vi "VIH UI - Controller for Property Pages.vi"(6 "cmd (update)":T2(ring)=enum."Update", 7 "SubPanel":refnum<vi>, 8 "error in":errorcluster, 9 "Params":string[](array[string]), 10 "Item Type":T3, 11 "Project Tree":T1) -> (0 "error out":errorcluster, 3 "dup Tree Refnum":T1)   [LabVIEW 2014]
doc: "::: VI Helpeks :::\nCopyright (c) 2000-2026 Konstantin Shifershteyn. All rights reserved."
uses:
  _VIH Project Manager.llb/VIH Project Tree Typedef - Tree Item Type.ctl
  _VIH Project Manager.llb/VIH Project Tree Typedef - Tree Refnum.ctl
  VIH UI Typedef - Property Page ExtCommand.ctl
panel:
  # "VI Helpeks\nCopyright (c) 2012-2026 Konstantin Shifershteyn"
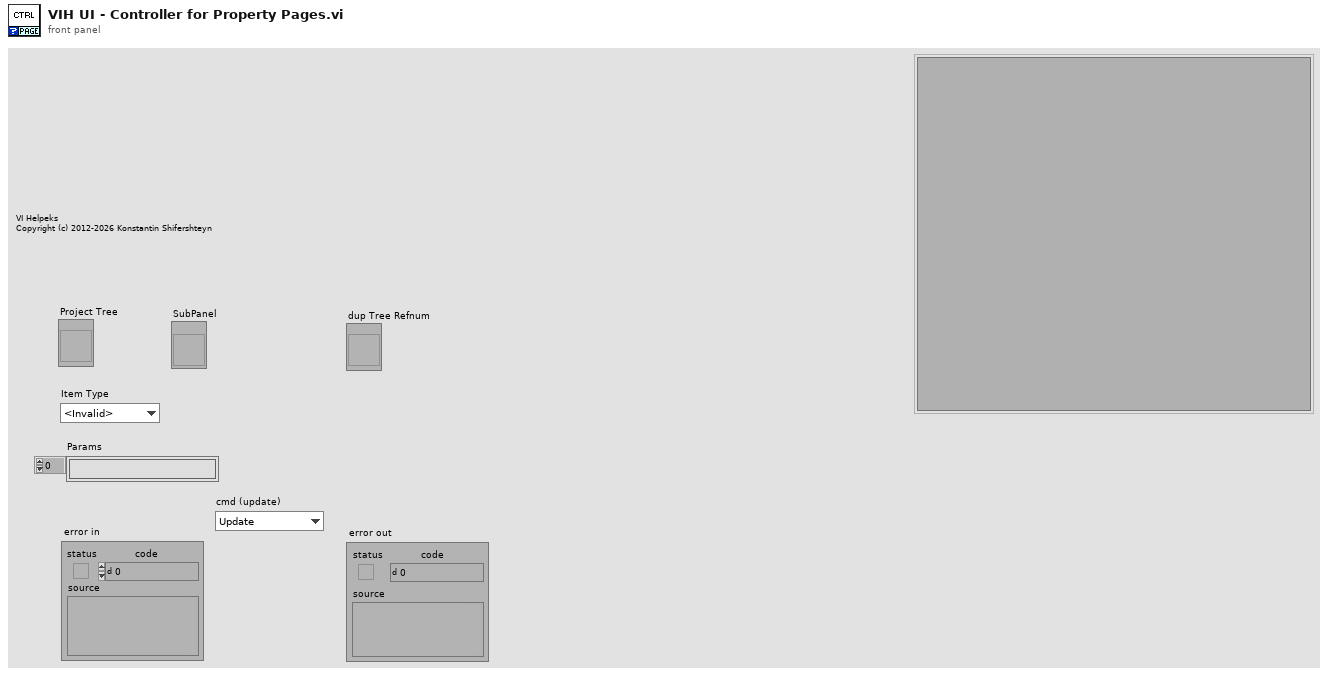
[diagram p1: front panel]
types:
  T1 = typedef "VIH Project Tree Typedef - Tree Refnum.ctl" = refnum<vi>
  T2 = enum16{"Open", "Close", "Update", "Set Category"}
  T3 = typedef "VIH Project Tree Typedef - Tree Item Type.ctl" = enum32{"<Invalid>", "Project", "Proj Files", "Proj Rules", "File Group", "Rule Group", "Any File", "LV Func", ".mnu", ".mnu (dyn)", ".vi", ".vi (dyn)", ".vit", ".vit (dyn)", ".ctl", ".ctl (dyn)", ".ctt", ".ctt (dyn)", "polyVI", "polyVI (dyn)", "expVI", "expVI (dyn)", "HTML", "PolyVI Inst"}
  T4 = typedef "VIH UI Typedef - Property Page ExtCommand.ctl" = cluster{"Action":string, "Project Tree":T1, "Params":string[]}
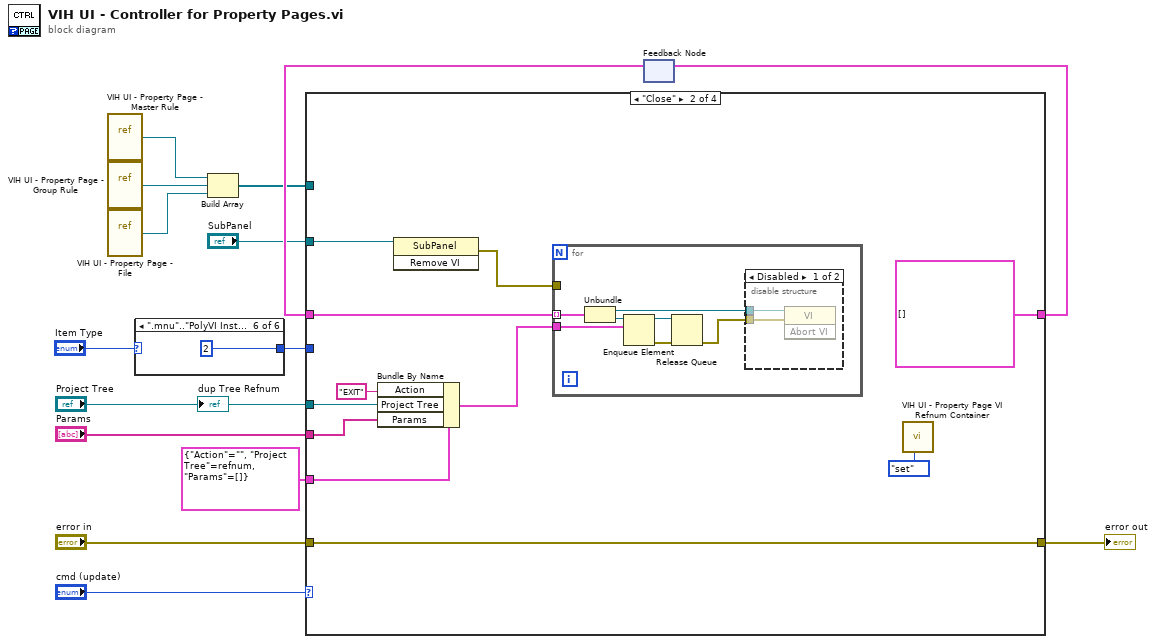
[diagram p0: block diagram]
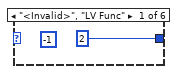
[diagram p2: hidden frame]
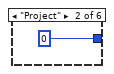
[diagram p3: hidden frame]
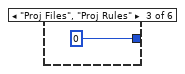
[diagram p4: hidden frame]
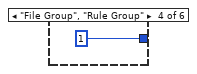
[diagram p5: hidden frame]
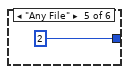
[diagram p6: hidden frame]
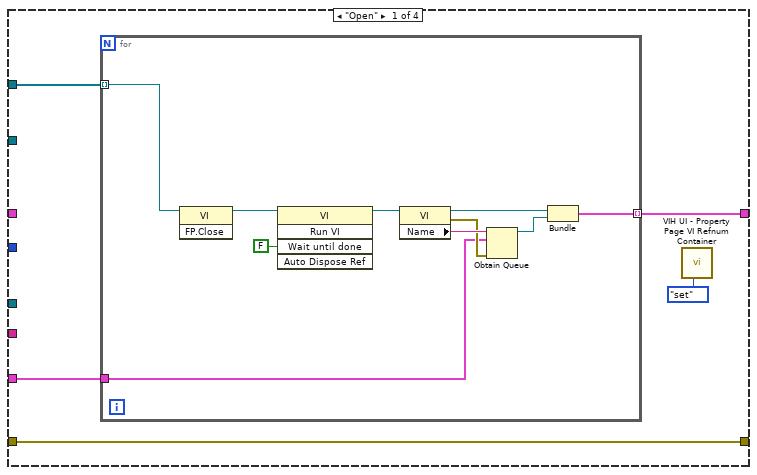
[diagram p7: hidden frame]
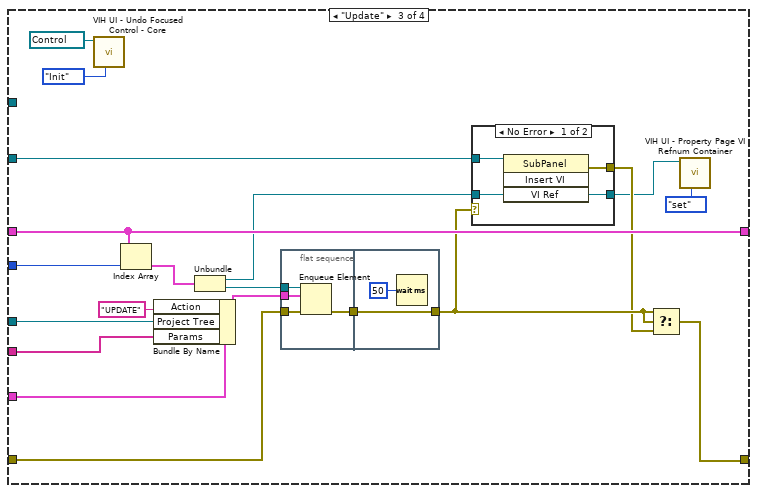
[diagram p9: hidden frame]
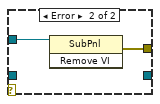
[diagram p10: hidden frame]
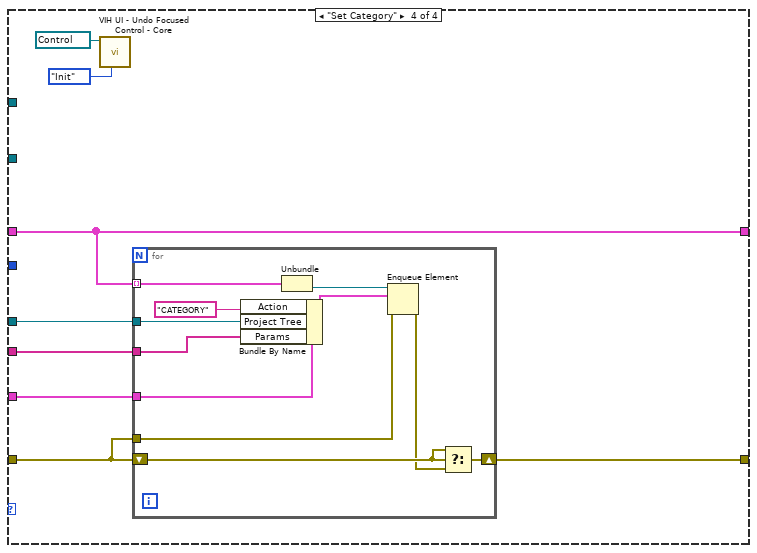
[diagram p11: hidden frame]
diagram:
  n1 = vi-ref "VIH UI - Property Page - Master Rule.vi"() -> (w7:refnum<vi>)
  n2 = vi-ref "VIH UI - Property Page - Group Rule.vi"() -> (w6:refnum<vi>)
  n3 = vi-ref "VIH UI - Property Page - File.vi"() -> (w5:refnum<vi>)
  n4 = case shown="\".mnu\"..\"PolyVI Inst\"" "Item Type" {
    tunnel: [2 0 0 1 2 2] -> w4
    frame "<Invalid>", "LV Func" {
      (unwired) -1
    }
    frame "Project" {
    }
    frame "Proj Files", "Proj Rules" {
    }
    frame "File Group", "Rule Group" {
    }
    frame "Any File" {
    }
    frame ".mnu".."PolyVI Inst" {
    }
  }
  n5 = Build Array(w7, w6, w5) -> (w2:refnum<vi>[])
  n6 = feedback #1() -> (w13:cluster{refnum<vi>, "queue out":refnum<queue>}[])  [unwired: 1 in]
  n7 = case shown="\"Close\"" "cmd (update)" {
    tunnel: [w26 cluster{refnum<vi>, "queue out":refnum<queue>}[] [] w76 w92] -> w14
    tunnel: w13 -> [_ w47 w76 w92]
    tunnel: "Params" -> [_ w42 w73 w95]
    tunnel: w4 -> [_ _ w70 _]
    tunnel: "error in" -> [w25 w46 w68 w91]
    tunnel: [w25 w46 w61 w90] -> w10
    tunnel: T4 {"Action"="", "Project Tree"=refnum, "Params"=[]} -> [w24 w45 w67 w94]
    tunnel: "Project Tree" -> [_ w43 w66 w93]
    tunnel: w2 -> [w23 _ _ _]
    tunnel: "SubPanel" -> [_ w39 w64 _]
    frame "Open" {
      n8 = for {
        tunnel: [w31] -> w26 mode=indexing
        tunnel: w24 -> [w29]
        tunnel: w23 -> [w28] mode=indexing
        n9 = invoke class="VI" method="FP.Close"(reference=w28) -> (reference out=w27:refnum<vi>)  [unwired: 2 in, 2 out]
        n10 = invoke class="VI" method="Run VI"(reference=w27, "Wait until done"=FALSE ("Wait Until Done")) -> (reference out=w35:refnum<vi>)  [unwired: 3 in, 4 out]
        n11 = property class="VI"(reference=w35) -> (reference out=w33:refnum<vi>, error out=w30:errorcluster, "Name"=w34:string)  [unwired: 1 in]
        n12 = Obtain Queue(name (unnamed)=w34, element data type=w29, error in (no error)=w30) -> (queue out=w32:refnum<queue>)  [unwired: 2 in, 2 out]
        n13 = Bundle(w33, "queue out"=w32) -> (w31:cluster{refnum<vi>, "queue out":refnum<queue>})  [unwired: 1 in]
      }
      n14 = call "VIH UI - Property Page VI Refnum Container.vi"("cmd (get)"=enum16{"get", "set"}."set") -> ()  [unwired: 9 in, 2 out]
    }
    frame "Close" {
      n15 = Bundle By Name(cluster=w45, "Action"="EXIT", "Project Tree"=w43, "Params"=w42) -> (w41:T4)
      n16 = invoke on="Invoke Node" class="SubPanel" method="Remove VI"(reference=w39) -> (error out=w38:errorcluster)  [unwired: 2 in, 2 out]
      n17 = for {
        tunnel: w47 -> [w54] mode=indexing
        tunnel: w41 -> [w48]
        tunnel: w38 -> [_]
        n18 = Unbundle(w54) -> (w50:refnum<vi>, "queue out"=w53:refnum<queue>)
        n19 = Enqueue Element(queue=w53, element=w48) -> (queue out=w52:refnum<queue>, error out=w51:errorcluster)  [unwired: 2 in, 1 out]
        n20 = Release Queue(queue=w52, error in (no error)=w51) -> (error out=w49:errorcluster)  [unwired: 1 in, 2 out]
        n21 = disable-structure shown="Disabled" {
          disable-tunnel: w50 -> [w56 _]
          disable-tunnel: w49 -> [w55 _]
          frame Disabled {
            n22 = invoke class="VI" method="Abort VI"(reference=w56, error in=w55) -> ()  [unwired: 1 in, 3 out]
          }
          frame Enabled {
          }
        }
      }
      n23 = call "VIH UI - Property Page VI Refnum Container.vi"("cmd (get)"=enum16{"get", "set"}."set") -> ()  [unwired: 9 in, 2 out]
    }
    frame "Update" {
      n24 = call "VIH UI - Undo Focused Control - Core.vi"("cmd (save)"=enum16{"Init", "status", "save", "undo", "redo"}."Init" ("cmd (click)"), "Ctl Refnum"=refnum<vi> refnum) -> ()  [unwired: 7 in, 3 out]
      n25 = Index Array(array=w76, index=w70) -> (element=w75:cluster{refnum<vi>, "queue out":refnum<queue>})
      n26 = Bundle By Name(cluster=w67, "Action"="UPDATE", "Project Tree"=w66, "Params"=w73) -> (w71:T4)
      n27 = Unbundle(w75) -> (w69:refnum<vi>, "queue out"=w74:refnum<queue>)
      n28 = flat-sequence {
        tunnel: w74 -> [w80]
        tunnel: w71 -> [w79]
        tunnel: w68 -> [w78]
        tunnel: [w77] -> w65
        tunnel: [w82] -> w63
        tunnel: w65 -> [w82]
        frame #0 {
          n29 = Enqueue Element(queue=w80, element=w79, error in (no error)=w78) -> (error out=w77:errorcluster)  [unwired: 1 in, 2 out]
        }
        frame #1 {
          n30 = Wait (ms)(milliseconds to wait=u32 50) -> ()  [unwired: 1 out]
        }
      }
      n31 = case shown="No Error" w63 {
        tunnel: w69 -> [w83 _]
        tunnel: [w85 w87] -> w62
        tunnel: w64 -> [w84 w86]
        tunnel: [w83 _] -> w58
        frame No Error {
          n32 = invoke on="Invoke Node" class="SubPanel" method="Insert VI"(reference=w84, "VI Ref"=w83) -> (error out=w85:errorcluster)  [unwired: 2 in, 3 out]
        }
        frame Error {
          n33 = invoke class="SubPnl" method="Remove VI"(reference=w86) -> (error out=w87:errorcluster)  [unwired: 2 in, 2 out]
        }
      }
      n34 = Select(t=w63, s=w63, f=w62) -> (s? t:f=w61:errorcluster)
      n35 = call "VIH UI - Property Page VI Refnum Container.vi"("cmd (get)"=enum16{"get", "set"}."set", "VI Refnum"=w58) -> ()  [unwired: 8 in, 2 out]
    }
    frame "Set Category" {
      n36 = call "VIH UI - Undo Focused Control - Core.vi"("cmd (save)"=enum16{"Init", "status", "save", "undo", "redo"}."Init" ("cmd (click)"), "Ctl Refnum"=refnum<vi> refnum) -> ()  [unwired: 7 in, 3 out]
      n37 = for {
        tunnel: w95 -> [w105]
        tunnel: w91 -> [w102]
        tunnel: w94 -> [w101]
        tunnel: w93 -> [w100]
        tunnel: w92 -> [w99] mode=indexing
        shift-right: [w96] -> w90
        shift-left: w91 -> [w98]
        n38 = Bundle By Name(cluster=w101, "Action"="CATEGORY", "Project Tree"=w100, "Params"=w105) -> (w103:T4)
        n39 = Unbundle(w99) -> ("queue out"=w106:refnum<queue>)  [unwired: 1 out]
        n40 = Enqueue Element(queue=w106, element=w103, error in (no error)=w102) -> (error out=w97:errorcluster)  [unwired: 1 in, 2 out]
        n41 = Select(t=w98, s=w98, f=w97) -> (s? t:f=w96:errorcluster)
      }
    }
  }
  "error out" <- w10
  n42 = feedback-in #1(w14) -> ()
  "dup Tree Refnum" <- "Project Tree"
